vi "P8_CleanUpDiagram.vi"(11 "Inputs":string[](array[string])) -> (2 "Output/Failure":string, 3 "CLI Process Return Code":i32)   [LabVIEW 2026]
doc: "Slice 1.1 probe: Open VI Reference, move the first node of the diagram to Left 2000, BD.CleanUp, read the node's Left again, close the reference."
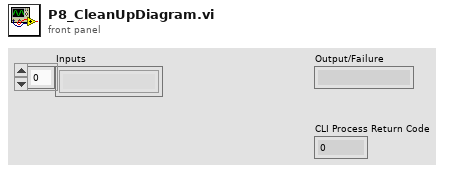
[diagram p1: front panel]
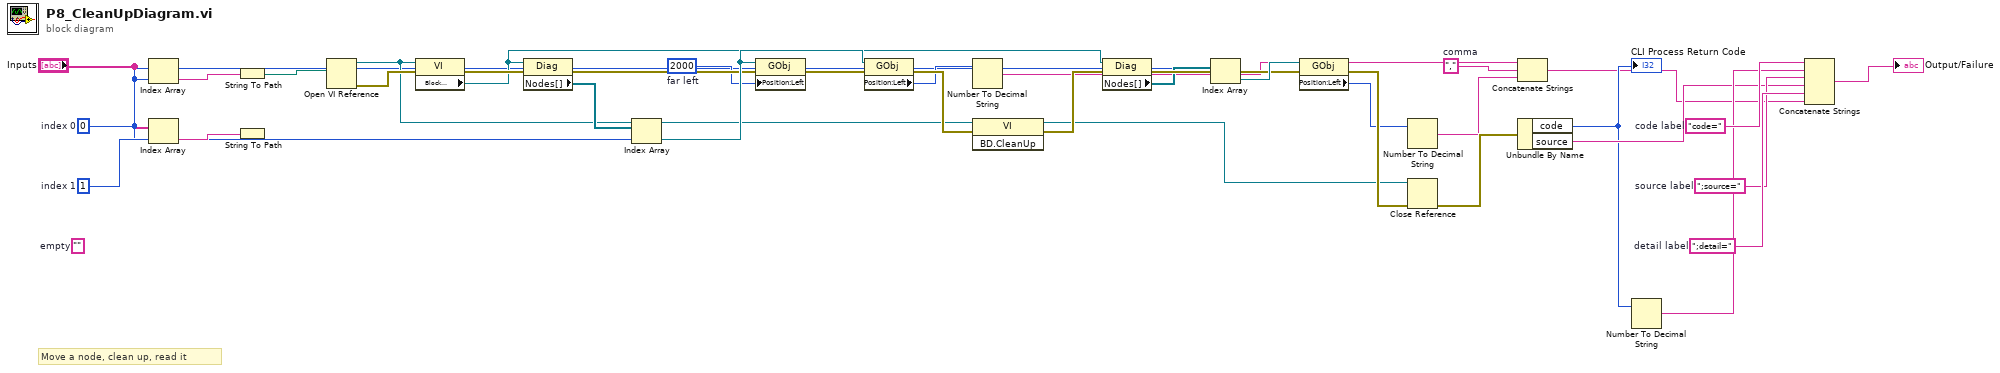
[diagram p0: block diagram]
diagram:
  w35 = ";detail="  # detail label
  w34 = ";source="  # source label
  w33 = "code="  # code label
  w12 = ","  # comma
  w11 = i16 2000  # far left
  (unwired) ""  # empty
  w3 = 1  # index 1
  w2 = 0  # index 0
  # "Move a node, clean up, read it"
  n1 = Index Array(array="Inputs", index=w2) -> (element=w4:string)
  n2 = Index Array(array="Inputs", index=w3) -> (element=w5:string)
  n3 = String To Path(string=w4) -> (path=w6:path)
  n4 = String To Path(string=w5) -> ()  [unwired: 1 out]
  n5 = Open VI Reference(vi path=w6) -> (vi reference=w7:refnum<vi>, error out=w8:errorcluster)  [unwired: 5 in]
  n6 = property class="VI"(reference=w7, error in=w8) -> (error out=w10:errorcluster, "Block Diagram"=w9:refnum<vi>)  [unwired: 1 out]
  n7 = property class="Diag"(reference=w9, error in=w10) -> (error out=w14:errorcluster, "Nodes[]"=w13:refnum<vi>[])  [unwired: 1 out]
  n8 = Index Array(array=w13, index=w2) -> (element=w15:refnum<vi>)
  n9 = property class="GObj"(reference=w15, error in=w14, "Position:Left"=w11) -> (error out=w16:errorcluster)  [unwired: 1 out]
  n10 = property class="GObj"(reference=w15, error in=w16) -> (error out=w18:errorcluster, "Position:Left"=w17:i32)  [unwired: 1 out]
  n11 = Number To Decimal String(number=w17) -> (decimal integer string=w19:string)  [unwired: 1 in]
  n12 = invoke class="VI" method="BD.CleanUp"(reference=w7, error in=w18) -> (reference out=w20:refnum<vi>, error out=w21:errorcluster)  [unwired: 1 in, 1 out]
  n13 = property class="Diag"(reference=w9, error in=w21) -> (error out=w23:errorcluster, "Nodes[]"=w22:refnum<vi>[])  [unwired: 1 out]
  n14 = Index Array(array=w22, index=w2) -> (element=w24:refnum<vi>)
  n15 = property class="GObj"(reference=w24, error in=w23) -> (error out=w26:errorcluster, "Position:Left"=w25:i32)  [unwired: 1 out]
  n16 = Number To Decimal String(number=w25) -> (decimal integer string=w27:string)  [unwired: 1 in]
  n17 = Close Reference(reference=w20, error in (no error)=w26) -> (error out=w29:errorcluster)
  n18 = Concatenate Strings(w19, w12, w27) -> (w28:string)
  n19 = Unbundle By Name(w29) -> ("code"=w30:i32, "source"=w31:string)
  "CLI Process Return Code" <- w30
  n20 = Number To Decimal String(number=w30) -> (decimal integer string=w32:string)  [unwired: 1 in]
  n21 = Concatenate Strings(w33, w32, w34, w31, w35, w28) -> (→"Output/Failure":string)
